vi "fix sync item names.vi"(11 "sync items in":T1[](array[typedef])) -> (3 "sync items out":T1[](array[typedef]))   [LabVIEW 2014, in "Shared Memory editor node.lvclass"]
uses:
  Shared Memory editor node.lvclass
  sync/sync item.ctl
  sync/sync mechanism.ctl
  module/configuration/Shared Memory configuration.lvclass
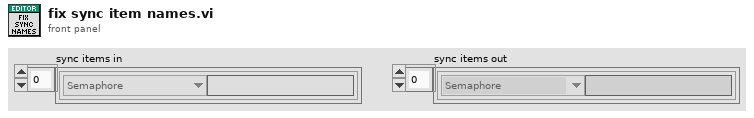
[diagram p1: front panel]
types:
  T1 = typedef "Shared Memory configuration.lvclass/sync item.ctl" = cluster{"mechanism":T2, "name":string}
  T2 = typedef "Shared Memory configuration.lvclass/sync mechanism.ctl" = enum16{"Semaphore"}
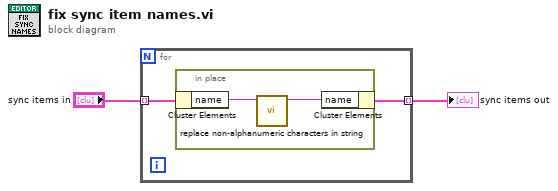
[diagram p0: block diagram]
diagram:
  n1 = for {
    tunnel: "sync items in" -> [w4] mode=indexing
    tunnel: [w3] -> w2 mode=indexing
    n2 = in-place {
      n3 = in-place-cluster #1(w4) -> ("name"=w6:string)
      n4 = call "replace non-alphanumeric characters in string.vi"("string in"=w6) -> ("string out"=w5:string)  [unwired: 10 in]
      n5 = in-place-cluster #1("name"=w5) -> (w3:T1)
    }
  }
  "sync items out" <- w2
